vi "Parse Load SA Range Setting.vi"(8 "error in (no error)":errorcluster caption="에러 입력(에러 없음)", 10 "문자열":string, 11 "Instrument Manager 입력":refnum<class "Instrument Manager.lvclass">) -> (0 "error out":errorcluster caption="에러 출력", 1 "SA Range Param":T1, 2 "Load SA Range Setting Param":T2, 3 "Instrument Manager 출력":refnum<class "Instrument Manager.lvclass">)   [LabVIEW 2023, in "Instrument Manager.lvclass"]
uses:
  Instrument Manager.lvclass
  Type Definition/SA Range Param.ctl
  Param Definition/Load SA Range Setting Param.ctl
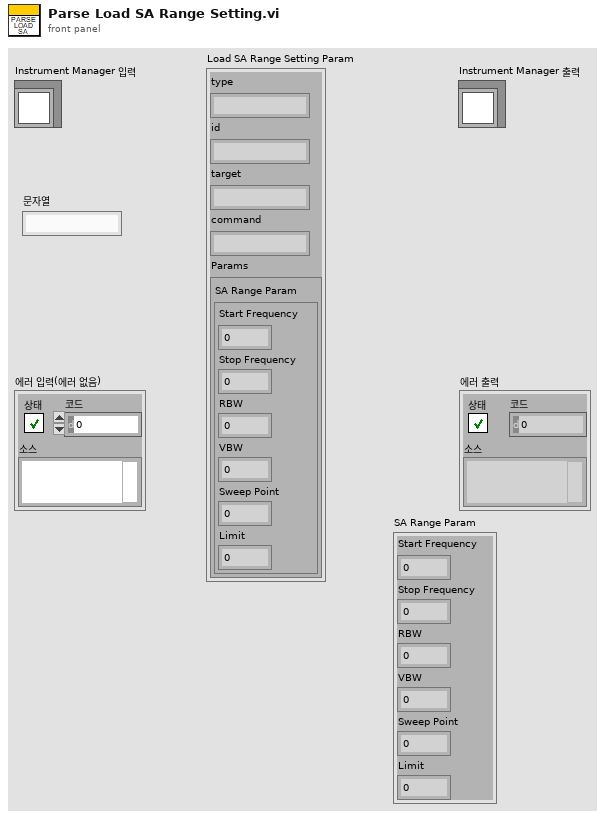
[diagram p1: front panel]
types:
  T1 = typedef "SA Range Param.ctl" = cluster{"Start Frequency":dbl, "Stop Frequency":dbl, "RBW":dbl, "VBW":dbl, "Sweep Point":u32, "Limit":dbl}
  T2 = typedef "Instrument Manager.lvclass/Load SA Range Setting Param.ctl" = cluster{"type":string, "id":string, "target":string, "command":string, "Params":cluster{"SA Range Param":T1}}
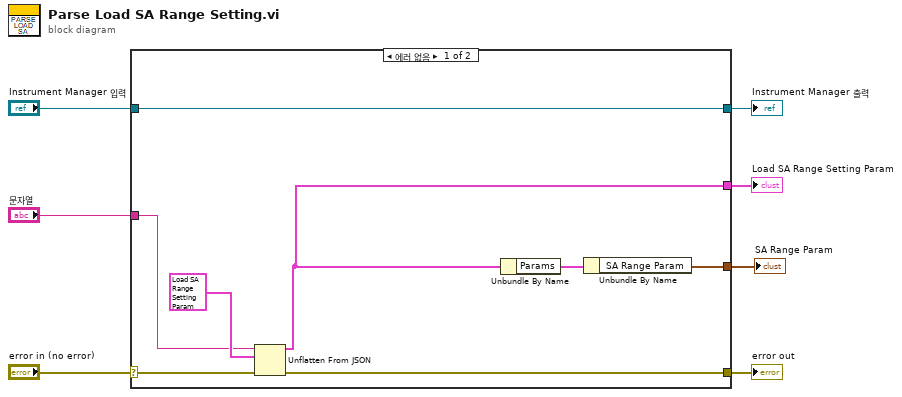
[diagram p0: block diagram]
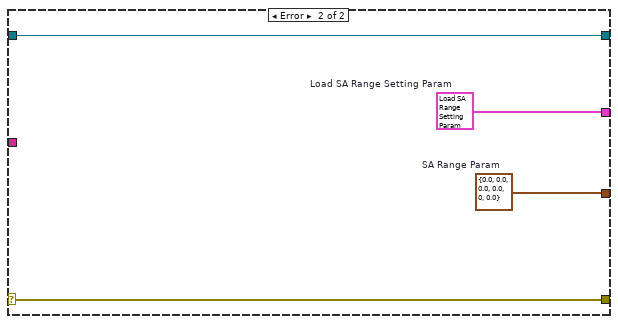
[diagram p2: hidden frame]
diagram:
  n1 = case shown="에러 없음" "error in (no error)" {
    selector: "error in (no error)" -> [w14 w19]
    tunnel: [w13 w19] -> w6
    tunnel: [w15 w18] -> w4
    tunnel: "Instrument Manager 입력" -> [w15 w18]
    tunnel: "문자열" -> [w11 _]
    tunnel: [w8 w16] -> w1
    tunnel: [w10 w17] -> w2
    frame No Error {
      n2 = Unflatten From JSON(JSON string=w11, type and defaults=T2 {"type"="", "id"="", "target"="", "command"="", "Params"={"SA Range Param"={"Start Frequency"=0.0, "Stop Frequency"=0.0, "RBW"=0.0, "VBW"=0.0, "Sweep Point"=0, "Limit"=0.0}}} ("Load SA Range Setting Param"), error in (no error)=w14) -> (value=w10:T2, error out=w13:errorcluster)  [unwired: 4 in]
      n3 = Unbundle By Name(w10) -> ("Params"=w9:cluster{"SA Range Param":T1})
      n4 = Unbundle By Name(w9) -> ("SA Range Param"=w8:T1)
    }
    frame Error {
      w16 = T1 {"Start Frequency"=0.0, "Stop Frequency"=0.0, "RBW"=0.0, "VBW"=0.0, "Sweep Point"=0, "Limit"=0.0}  # SA Range Param
      w17 = T2 {"type"="", "id"="", "target"="", "command"="", "Params"={"SA Range Param"={"Start Frequency"=0.0, "Stop Frequency"=0.0, "RBW"=0.0, "VBW"=0.0, "Sweep Point"=0, "Limit"=0.0}}}  # Load SA Range Setting Param
    }
  }
  "error out" <- w6
  "Instrument Manager 출력" <- w4
  "Load SA Range Setting Param" <- w2
  "SA Range Param" <- w1
